vi "Sous_VI_correcteur_encodeur.vi"(8 "Pulse Droit":dbl, 9 "Pulse Gauche":dbl, 11 "Duty ref":dbl) -> (0 "Duty Droit":dbl, 3 "Duty Gauche":dbl)   [LabVIEW 2017]
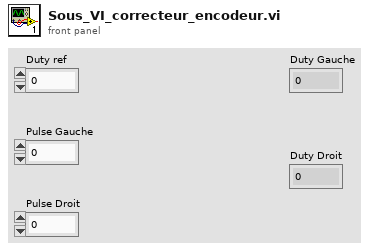
[diagram p1: front panel]
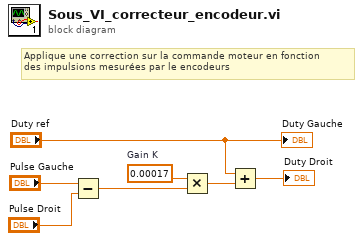
[diagram p0: block diagram]
diagram:
  w4 = 0.00017  # Gain K
  # "Applique une correction sur la commande moteur en fonction\ndes impulsions mesurées par le encodeurs"
  n1 = Subtract(x="Pulse Gauche", y="Pulse Droit") -> (x-y=w2:dbl)
  n2 = Multiply(x=w4, y=w2) -> (x*y=w1:dbl)
  n3 = Add(x="Duty ref", y=w1) -> (x+y=→"Duty Droit":dbl)
  "Duty Gauche" <- "Duty ref"
